vi "MethodSignatureDialogvi.vi"() -> (2 "Cancelled":bool)   [LabVIEW 2020, in "ClassWriterNative.lvclass"]
uses:
  ClassWriterNative.lvclass
panel:
  in  "Help":bool
  out "ProductPicture":picture
  in  "_ShowContextHelp":bool
  in  "_UpdateSignature":bool caption="Update this signature"
  in  "_InsertTag":bool caption="Insert tag"
  out "_TagPreview":string caption="Tag preview"
  in  "_SelectTagToAdd":T1(ring) caption="Select a tag to a cursor"
  in  "_SignatureName":string caption="Signature name"
  in  "_ModifySignature":bool caption="Modify signature"
  in  "_RemoveSignature":bool caption="Remove signature"
  in  "_Cancel":bool
  in  "_Done":bool
  in  "_AddSignature":bool caption="Add this signature"
  in  "_Signatures":i32[](listbox) caption="Signatures"
  in  "_SignatureText":string caption="Signature text"
  out "error out":errorcluster
  in  "error in":errorcluster
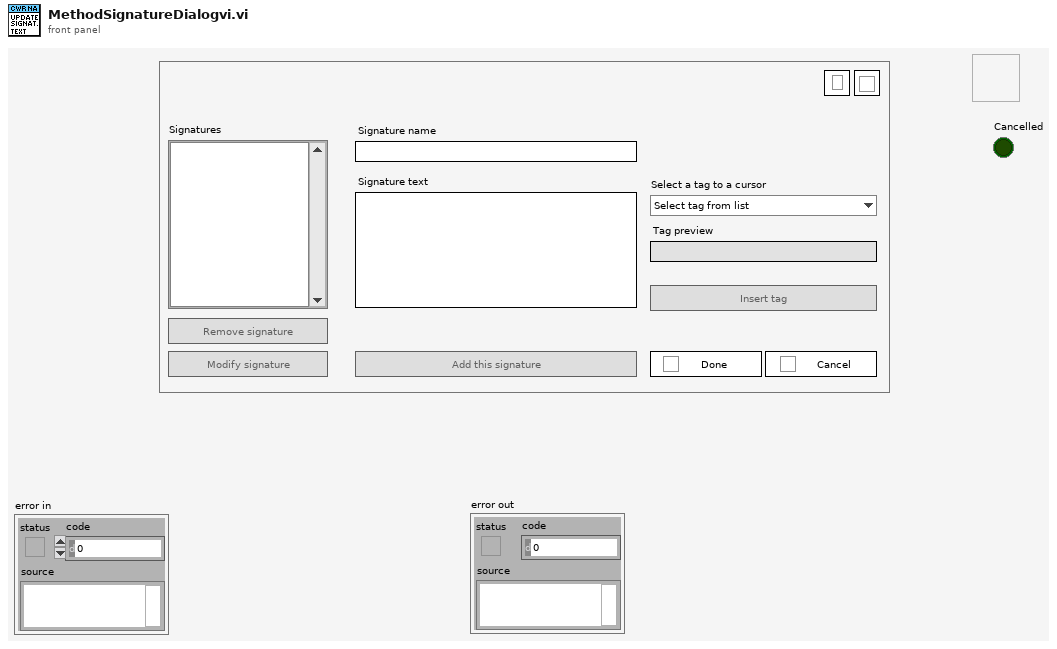
[diagram p1: front panel]
types:
  T1 = enum16{"Select tag from list", "<Date>", "<DateTime>", "<User>", "<LvVersion>"}
  T2 = cluster{"Cancelled":bool, "SignatureName":string[], "SignatureText":string[], "Current":i32}
  T3 = cluster{"SignatureName":string[], "SignatureText":string[], "Current":i32}
  T4 = cluster{"SignatureName":string[], "SignatureText":string[], i32}
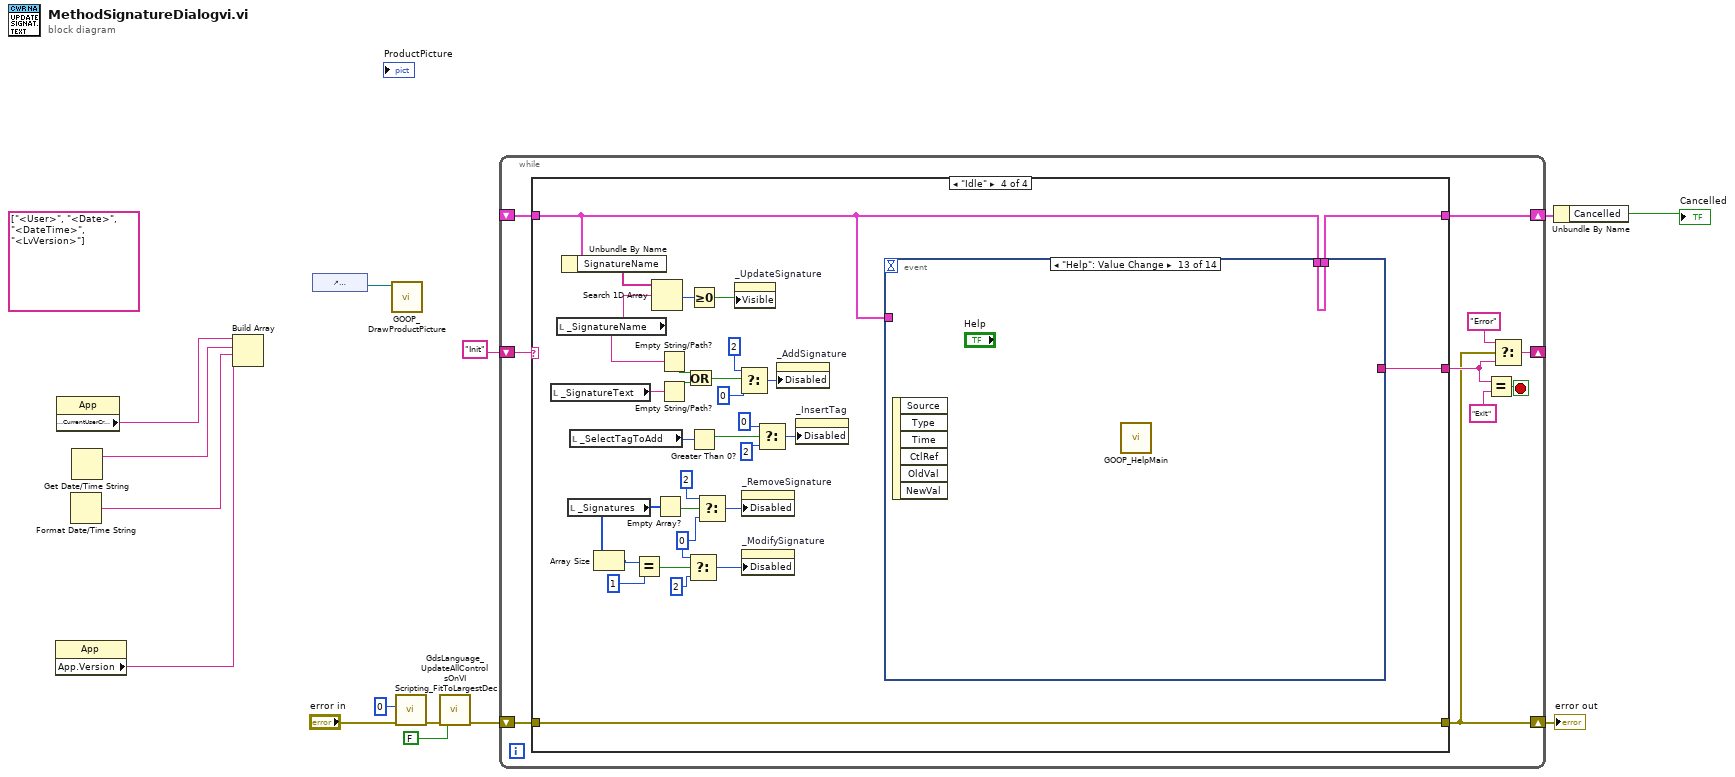
[diagram p0: block diagram]
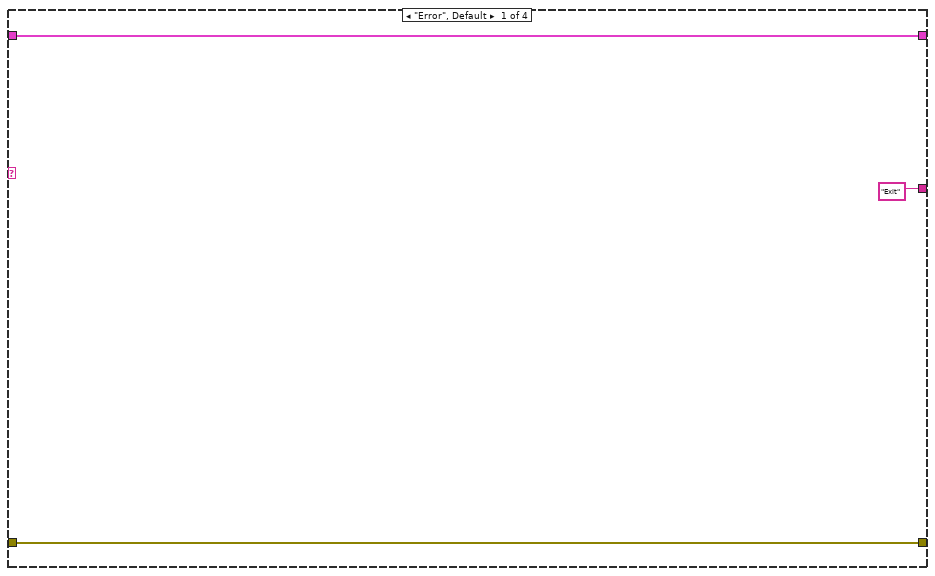
[diagram p2: hidden frame]
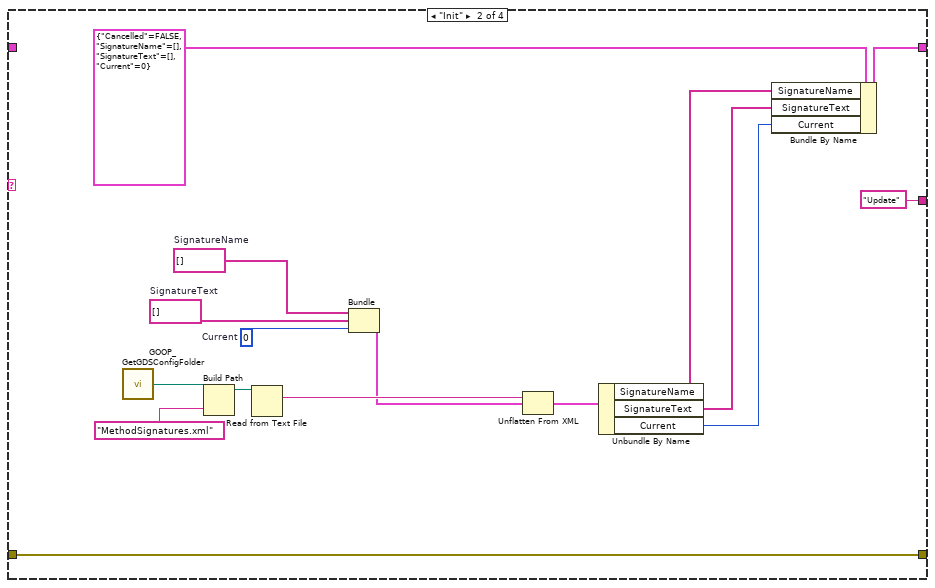
[diagram p3: hidden frame]
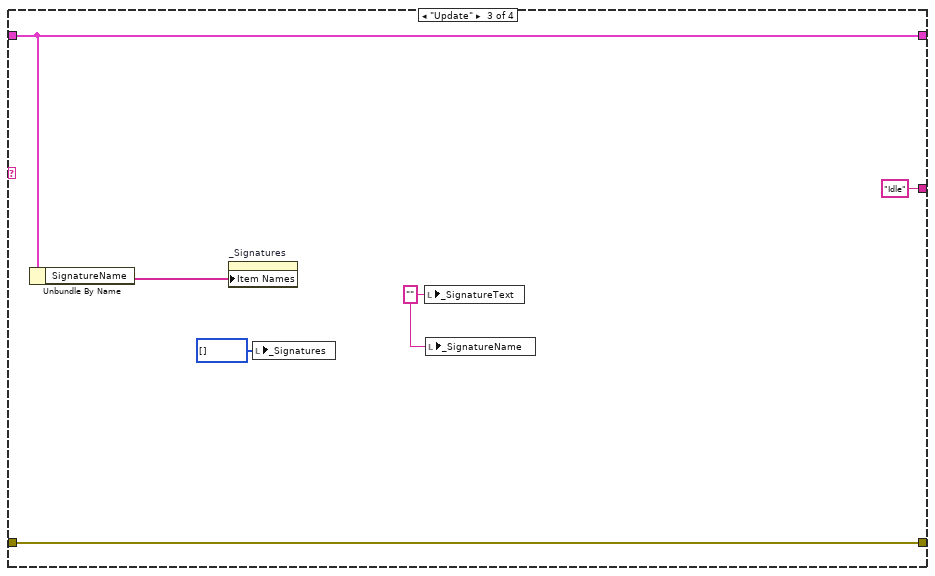
[diagram p4: hidden frame]
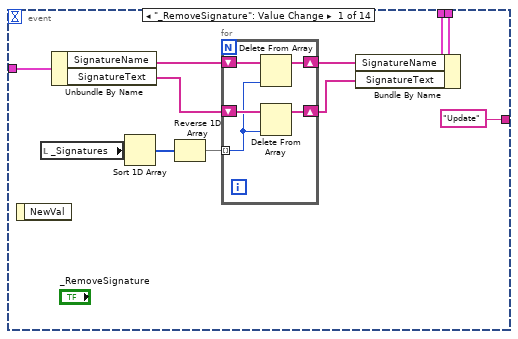
[diagram p5: hidden frame]
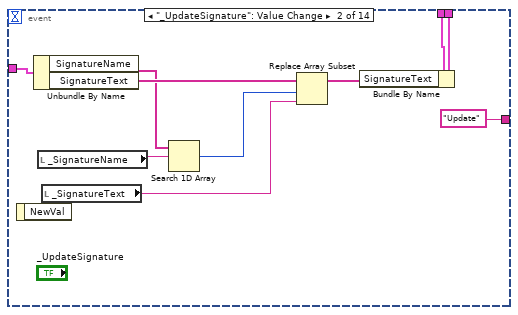
[diagram p6: hidden frame]
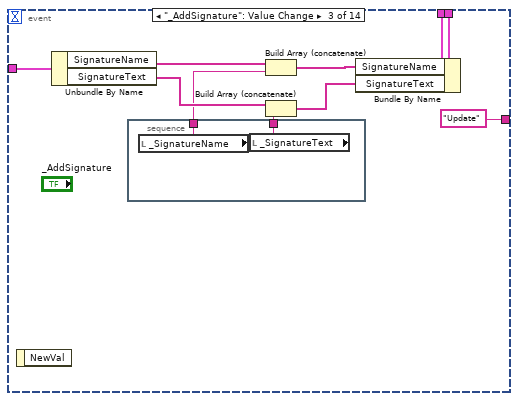
[diagram p7: hidden frame]
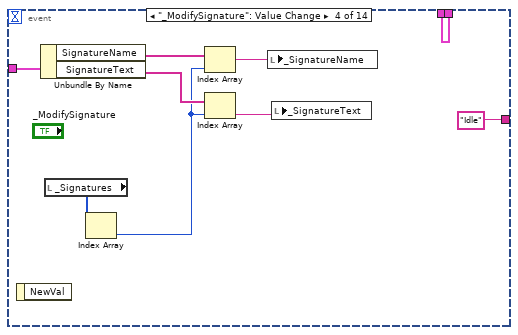
[diagram p8: hidden frame]
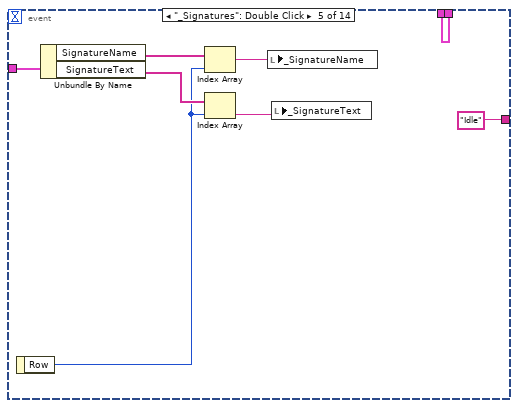
[diagram p9: hidden frame]
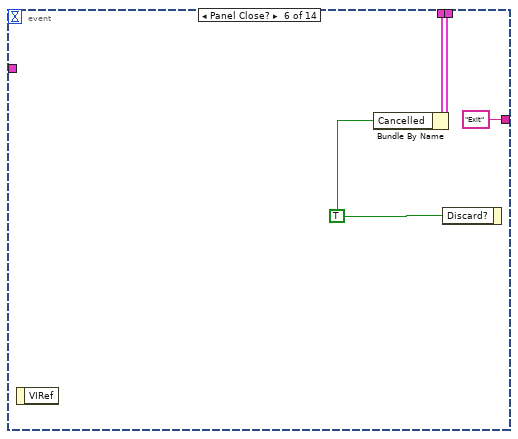
[diagram p10: hidden frame]
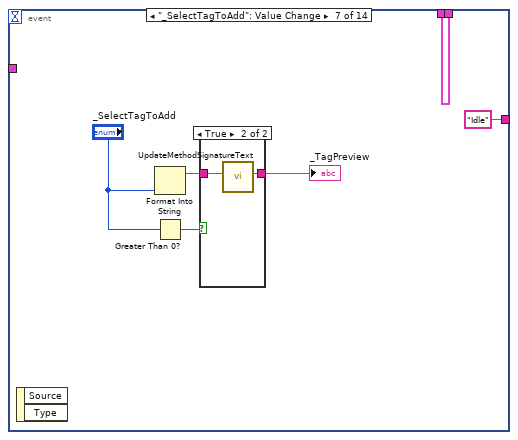
[diagram p11: hidden frame]
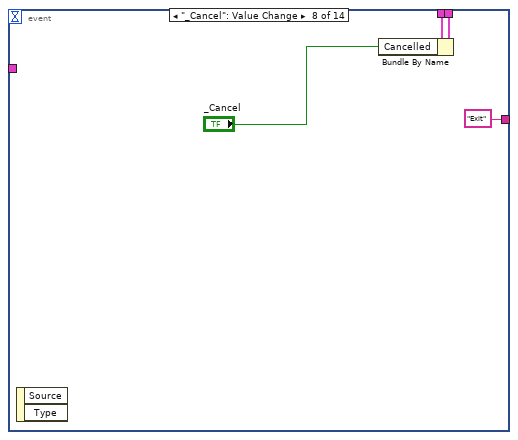
[diagram p13: hidden frame]
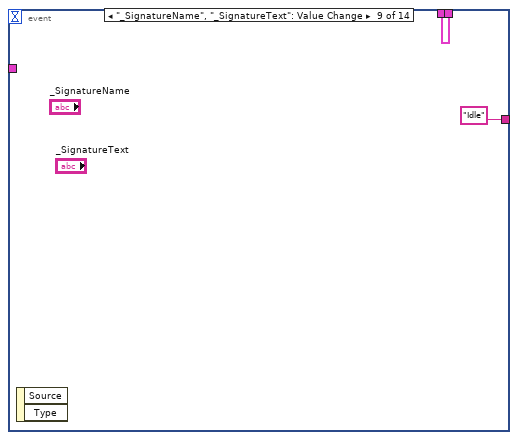
[diagram p14: hidden frame]
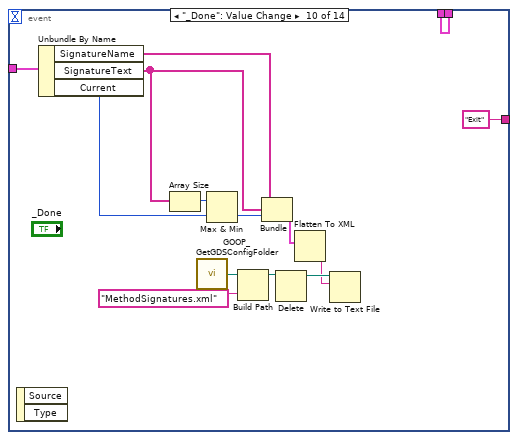
[diagram p15: hidden frame]
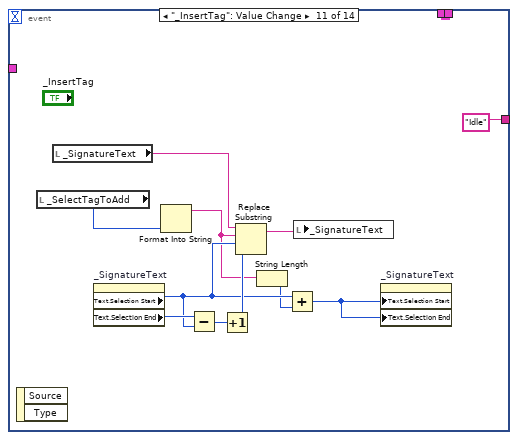
[diagram p16: hidden frame]
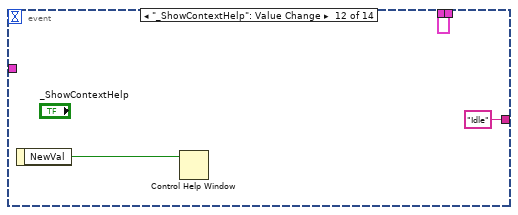
[diagram p17: hidden frame]
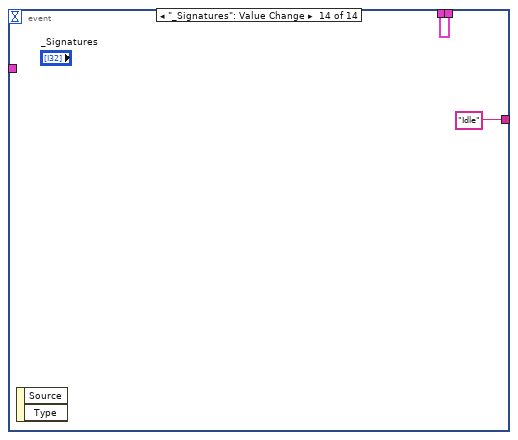
[diagram p18: hidden frame]
diagram:
  (unwired) string[] ["<User>", "<Date>", "<DateTime>", "<LvVersion>"]
  n1 = property class="App"() -> ("App.Version"=w11:string)  [unwired: 2 in, 2 out]
  n2 = property class="App"() -> ("App.CurrentUserCredential"=w14:string)  [unwired: 2 in, 2 out]
  n3 = Format Date/Time String() -> (date/time string=w12:string)  [unwired: 3 in]
  n4 = Get Date/Time String() -> (date string=w13:string)  [unwired: 3 in, 1 out]
  n5 = Build Array(w14, w13, w12, w11) -> ()  [unwired: 1 out]
  n6 = control-ref of="ProductPicture"() -> (w4:refnum<vi>)
  n7 = call "GOOP_DrawProductPicture.vi"("ProductPictureControl"=w4) -> ()  [unwired: 10 in, 1 out]
  n8 = call "Scripting_FitToLargestDec.vi"("error in (no error)"="error in", "border spacing (2 px)"=0) -> ("error out"=w1:errorcluster)  [unwired: 4 in, 1 out]
  n9 = call "GdsLanguage_UpdateAllControlsOnVI.vi"("error in (no error)"=w1, "CreateLanguageFile(Use this to create a languageFile)"=FALSE) -> ("error out"=w6:errorcluster)  [unwired: 16 in, 1 out]
  n10 = while {
    shift-right: [w17] -> w7
    shift-left: w6 -> [w24]
    shift-right: [w22] -> _
    shift-left: "Init" -> [w23]
    shift-right: [w16] -> w9
    shift-left: _ -> [w15]
    stop <- w21 stop-if-true
    n11 = case shown="\"Idle\"" w23 {
      tunnel: w24 -> [w27 w42 w47 w77]
      tunnel: [w27 w42 w47 w77] -> w17
      tunnel: ["Exit" "Update" "Idle" w78] -> w18
      tunnel: [w25 w40 w48 w79] -> w16
      tunnel: w15 -> [w25 _ w48 w66]
      frame "Error", Default {
      }
      frame "Init" {
        w35 = string[] []  # SignatureText
        w36 = string[] []  # SignatureName
        w33 = 0  # Current
        n12 = call "GOOP_GetGDSConfigFolder.vi"() -> ("GDSFolderPath"=w39:path)
        n13 = Build Path(base path=w39, name or relative path="MethodSignatures.xml") -> (appended path=w38:path)
        n14 = Read from Text File(file (use dialog)=w38) -> (text=w37:string)  [unwired: 3 in, 3 out]
        n15 = Bundle("SignatureName"=w36, "SignatureText"=w35, "Current"=w33) -> (w34:T3)  [unwired: 1 in]
        n16 = Unflatten From XML(xml string=w37, type=w34) -> (value=w32:T3)  [unwired: 1 in, 1 out]
        n17 = Unbundle By Name(w32) -> ("SignatureName"=w31:string[], "SignatureText"=w30:string[], "Current"=w29:i32)
        n18 = Bundle By Name(cluster=T2 {"Cancelled"=FALSE, "SignatureName"=[], "SignatureText"=[], "Current"=0}, "SignatureName"=w31, "SignatureText"=w30, "Current"=w29) -> (w40:T2)
      }
      frame "Update" {
        w44 = "" ("_SignatureText")
        n19 = Unbundle By Name(w48) -> ("SignatureName"=w46:string[])
        n20 = property on="_Signatures" class="LstBox (strict)"("Item Names"=w46) -> ()  [unwired: 2 in, 2 out]
        n21 = local write "_Signatures"(i32[] [] ("_Signatures")) -> ()
        n22 = local write "_SignatureText"(w44) -> ()
        n23 = local write "_SignatureName"(w44) -> ()
      }
      frame "Idle" {
        w69 = u8 0 ("f")
        n24 = local read "_SignatureText"() -> (w61:string)
        n25 = local read "_SignatureName"() -> (w62:string)
        n26 = Unbundle By Name(w66) -> ("SignatureName"=w65:string[])
        n27 = local read "_Signatures"() -> (w73:i32[])
        n28 = local read "_SelectTagToAdd"() -> (w54:T1)
        n29 = Array Size(array=w73) -> (size(s)=w72:i32)
        n30 = Equal?(x=w72, y=1) -> (x = y?=w68:bool)
        n31 = Search 1D Array(1D array=w65, element=w62) -> (index of element=w64:i32)  [unwired: 1 in]
        n32 = Empty Array?(array=w73) -> (empty?=w76:bool)
        n33 = Empty String/Path?(string/path=w62) -> (empty?=w60:bool)
        n34 = Empty String/Path?(string/path=w61) -> (empty?=w59:bool)
        n35 = Or(x=w60, y=w59) -> (x .or. y?=w56:bool)
        n36 = Select(t=w69, s=w68, f=u8 2) -> (s? t:f=w67:u8)
        n37 = Greater Or Equal To 0?(x=w64) -> (x >= 0?=w63:bool)
        n38 = Greater Than 0?(x=w54) -> (x > 0?=w52:bool)
        n39 = Select(t=u8 2 ("Disabled"), s=w76, f=w69) -> (s? t:f=w75:u8)
        n40 = property on="_UpdateSignature" class="Bool"("Visible"=w63) -> ()  [unwired: 2 in, 2 out]
        n41 = Select(t=u8 2 ("Disabled"), s=w56, f=u8 0) -> (s? t:f=w55:u8)
        n42 = property on="_RemoveSignature" class="Bool"("Disabled"=w75) -> ()  [unwired: 2 in, 2 out]
        n43 = property on="_ModifySignature" class="Bool"("Disabled"=w67) -> ()  [unwired: 2 in, 2 out]
        n44 = Select(t=u8 0 ("f"), s=w52, f=u8 2) -> (s? t:f=w50:u8)
        n45 = property on="_AddSignature" class="Bool"("Disabled"=w55) -> ()  [unwired: 2 in, 2 out]
        n46 = property on="_InsertTag" class="Bool"("Disabled"=w50) -> ()  [unwired: 2 in, 2 out]
        n47 = event shown="[12] \"Help\": Value Change" {
          selector: _ -> [_ _ _ _ _ _ _ _ _ _ _ _ _ _]
          dyn-events: _ -> [_ _ _ _ _ _ _ _ _ _ _ _ _ _]
          timeout: _ -> [_ _ _ _ _ _ _ _ _ _ _ _ _ _]
          tunnel: w66 -> [w89 w104 w114 w118 w128 w137 w142 w150 w152 w166 w178 w181 w182 w184]
          tunnel: [w88 w103 w113 w118 w128 w136 w142 w149 w152 w166 w178 w181 w182 w184] -> w79
          tunnel: ["Update" "Update" "Update" "Idle" "Idle" "Exit" "Idle" "Exit" "Idle" "Exit" "Idle" "Idle" _ "Idle"] -> w78
          tunnel: w66 -> [w87 w102 w112 w125 w134 _ _ _ _ w165 _ _ _ _]
          event "_RemoveSignature": Value Change {
            n48 = event-data() -> ()  [unwired: 1 in, 1 out]
            n49 = local read "_Signatures"() -> (w82:i32[])
            n50 = Unbundle By Name(w87) -> ("SignatureName"=w86:string[], "SignatureText"=w84:string[])
            n51 = Sort 1D Array(array=w82) -> (sorted array=w81:i32[])
            n52 = Reverse 1D Array(array=w81) -> (reversed array=w80:i32[])
            n53 = for {
              tunnel: w80 -> [w91] mode=indexing
              shift-right: [w92] -> w83
              shift-left: w84 -> [w93]
              shift-right: [w94] -> w85
              shift-left: w86 -> [w95]
              n54 = Delete From Array(array=w95, index=w91) -> (array with subset deleted=w94:string[])  [unwired: 1 in, 1 out]
              n55 = Delete From Array(array=w93, index=w91) -> (array with subset deleted=w92:string[])  [unwired: 1 in, 1 out]
            }
            n56 = Bundle By Name(cluster=w89, "SignatureName"=w85, "SignatureText"=w83) -> (w88:T2)
          }
          event "_UpdateSignature": Value Change {
            n57 = event-data() -> ()  [unwired: 1 in, 1 out]
            n58 = Unbundle By Name(w102) -> ("SignatureName"=w99:string[], "SignatureText"=w101:string[])
            n59 = local read "_SignatureName"() -> (w98:string)
            n60 = local read "_SignatureText"() -> (w96:string)
            n61 = Search 1D Array(1D array=w99, element=w98) -> (index of element=w97:i32)  [unwired: 1 in]
            n62 = Replace Array Subset(array=w101, new element=w96, index=w97) -> (w100:string[])
            n63 = Bundle By Name(cluster=w104, "SignatureText"=w100) -> (w103:T2)
          }
          event "_AddSignature": Value Change {
            n64 = event-data() -> ()  [unwired: 1 in, 1 out]
            n65 = Unbundle By Name(w112) -> ("SignatureName"=w111:string[], "SignatureText"=w109:string[])
            n66 = stacked-sequence {
              tunnel: [w117] -> w107
              tunnel: [w116] -> w106
              frame #0 {
                n67 = local read "_SignatureName"() -> (w117:string)
                n68 = local read "_SignatureText"() -> (w116:string)
              }
            }
            n69 = Build Array (concatenate)(w111, w107) -> (w110:string[])
            n70 = Build Array (concatenate)(w109, w106) -> (w108:string[])
            n71 = Bundle By Name(cluster=w114, "SignatureName"=w110, "SignatureText"=w108) -> (w113:T2)
          }
          event "_ModifySignature": Value Change {
            n72 = event-data() -> ()  [unwired: 1 in, 1 out]
            n73 = Unbundle By Name(w125) -> ("SignatureName"=w124:string[], "SignatureText"=w123:string[])
            n74 = local read "_Signatures"() -> (w126:i32[])
            n75 = Index Array(array=w126) -> (element=w122:i32)  [unwired: 1 in]
            n76 = Index Array(array=w124, index=w122) -> (element=w120:string)
            n77 = Index Array(array=w123, index=w122) -> (element=w121:string)
            n78 = local write "_SignatureName"(w120) -> ()
            n79 = local write "_SignatureText"(w121) -> ()
          }
          event "_Signatures": Double Click {
            n80 = event-data() -> ("Row"=w127:i32)  [unwired: 1 in]
            n81 = Unbundle By Name(w134) -> ("SignatureName"=w133:string[], "SignatureText"=w132:string[])
            n82 = Index Array(array=w133, index=w127) -> (element=w130:string)
            n83 = Index Array(array=w132, index=w127) -> (element=w131:string)
            n84 = local write "_SignatureName"(w130) -> ()
            n85 = local write "_SignatureText"(w131) -> ()
          }
          event Panel Close? {
            w135 = TRUE ("Discard?")
            n86 = event-data() -> ()  [unwired: 1 in, 1 out]
            n87 = Bundle By Name(cluster=w137, "Cancelled"=w135) -> (w136:T2)
            n88 = event-data("Discard?"=w135) -> ()  [unwired: 1 in, 1 out]
          }
          event "_SelectTagToAdd": Value Change {
            n89 = event-data() -> ()  [unwired: 1 in, 2 out]
            n90 = Format Into String("_SelectTagToAdd") -> (resulting string=w144:string)  [unwired: 3 in, 1 out]
            n91 = Greater Than 0?(x="_SelectTagToAdd") -> (x > 0?=w139:bool)
            n92 = case shown="True" w139 {
              tunnel: w144 -> [_ w146]
              tunnel: [_ w145] -> w143
              frame False {
              }
              frame True {
                n93 = call "UpdateMethodSignatureText.vi"("TagCodedStringIn"=w146) -> ("StringOut"=w145:string)  [unwired: 10 in]
              }
            }
            "_TagPreview" <- w143
          }
          event "_Cancel": Value Change {
            n94 = event-data() -> ()  [unwired: 1 in, 2 out]
            n95 = Bundle By Name(cluster=w150, "Cancelled"="_Cancel") -> (w149:T2)
          }
          event "_SignatureName", "_SignatureText": Value Change {
            n96 = event-data() -> ()  [unwired: 1 in, 2 out]
          }
          event "_Done": Value Change {
            n97 = event-data() -> ()  [unwired: 1 in, 2 out]
            n98 = Unbundle By Name(w165) -> ("SignatureName"=w162:string[], "SignatureText"=w160:string[], "Current"=w159:i32)
            n99 = Array Size(array=w160) -> (size(s)=w161:i32)
            n100 = call "GOOP_GetGDSConfigFolder.vi"() -> ("GDSFolderPath"=w163:path)
            n101 = Max & Min(x=w161, y=w159) -> (min(x,y)=w158:i32)  [unwired: 1 out]
            n102 = Build Path(base path=w163, name or relative path="MethodSignatures.xml") -> (appended path=w156:path)
            n103 = Bundle("SignatureName"=w162, "SignatureText"=w160, w158) -> (w157:T4)  [unwired: 1 in]
            n104 = Delete(path (use dialog)=w156) -> (deleted path=w155:path)  [unwired: 4 in, 2 out]
            n105 = Flatten To XML(6:w157) -> (2:w154:string)
            n106 = Write to Text File(file (use dialog)=w155, text=w154) -> ()  [unwired: 2 in, 3 out]
          }
          event "_InsertTag": Value Change {
            n107 = event-data() -> ()  [unwired: 1 in, 2 out]
            n108 = local read "_SelectTagToAdd"() -> (w172:T1)
            n109 = local read "_SignatureText"() -> (w176:string)
            n110 = property on="_SignatureText" class="Str"() -> ("Text.Selection Start"=w170:u32, "Text.Selection End"=w175:u32)  [unwired: 2 in, 2 out]
            n111 = Format Into String(w172) -> (resulting string=w169:string)  [unwired: 3 in, 1 out]
            n112 = Subtract(x=w175, y=w170) -> (x-y=w174:u32)
            n113 = Increment(x=w174) -> (x+1=w173:u32)
            n114 = Replace Substring(2:w173, 3:w170, 4:w169, 5:w176) -> (1:w171:string)  [unwired: 1 out]
            n115 = String Length(string=w169) -> (length=w168:i32)
            n116 = Add(x=w170, y=w168) -> (x+y=w167:u32)
            n117 = local write "_SignatureText"(w171) -> ()
            n118 = property on="_SignatureText" class="Str"("Text.Selection Start"=w167, "Text.Selection End"=w167) -> ()  [unwired: 2 in, 2 out]
          }
          event "_ShowContextHelp": Value Change {
            n119 = event-data() -> ("NewVal"=w179:bool)  [unwired: 1 in]
            n120 = Control Help Window(1:w179) -> ()  [unwired: 1 in]
          }
          event "Help": Value Change {
            n121 = event-data() -> ()  [unwired: 1 in, 6 out]
            n122 = call "GOOP_HelpMain.vi"() -> ()  [unwired: 12 in]
          }
          event "_Signatures": Value Change {
            n123 = event-data() -> ()  [unwired: 1 in, 2 out]
          }
        }
      }
    }
    n124 = Equal?(x=w18, y="Exit") -> (x = y?=w21:bool)
    n125 = Select(t="Error", s=w17, f=w18) -> (s? t:f=w22:string)
  }
  "error out" <- w7
  n126 = Unbundle By Name(w9) -> ("Cancelled"=→"Cancelled":bool)
